vi "Start Writer.vi"(8 "error in (no error)":errorcluster, 11 "CAN RW CANsub in":refnum<class "CAN RW CANsub.lvclass">) -> (0 "error out":errorcluster, 3 "CAN RW CANsub out":refnum<class "CAN RW CANsub.lvclass">)   [LabVIEW 2021, in "CAN RW CANsub.lvclass"]
uses:
  CAN RW CANsub.lvclass
  CAN RW CANsub.lvclass/CAN RW CANsub.ctl
  CANsub/c_client/api/CANsub_Channel/CANsub_Channel.lvclass
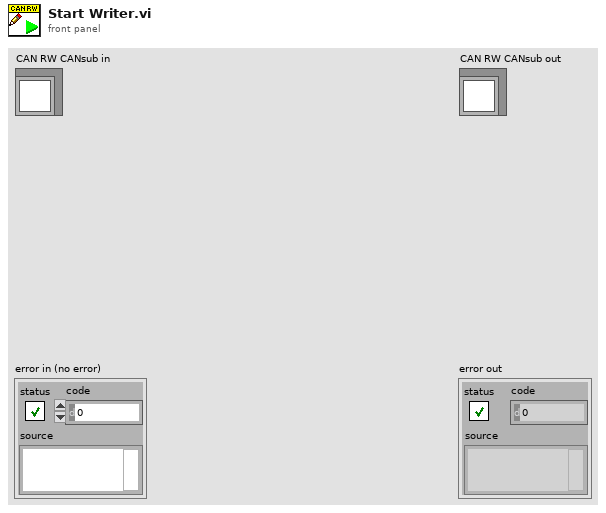
[diagram p1: front panel]
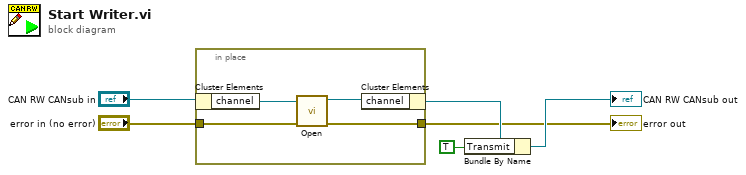
[diagram p0: block diagram]
diagram:
  n1 = in-place {
    in-place-border: "error in (no error)" -> [w9]
    in-place-border: [w7] -> w1
    n2 = in-place-cluster #1("CAN RW CANsub in") -> ("channel"=w10:refnum<class "CANsub_Channel.lvclass">)
    n3 = call-dynamic "Open.vi"("error in (no error)"=w9, "channel in"=w10) -> ("error out"=w7:errorcluster, "channel out"=w8:refnum<class "CANsub_Channel.lvclass">)  [unwired: 8 in]
    n4 = in-place-cluster #1("channel"=w8) -> (w4:refnum<class "CAN RW CANsub.lvclass">)
  }
  "error out" <- w1
  n5 = Bundle By Name(cluster=w4, "Transmit"=TRUE) -> (→"CAN RW CANsub out":refnum<class "CAN RW CANsub.lvclass">)
